vi "Test Load Day.vi"(8 "error in":errorcluster, 10 "Work Folder":path, 11 "Test Data Folder":path) -> (0 "error out":errorcluster, 2 "Report":string, 3 "Passed":bool)   [LabVIEW 2026]
doc: "Tests Load Day.vi on the schema-v2 sample data (Test Data\\Samples, copied into a new case folder and opened with Initialize Stores.vi). The day shown is 2025-10-06, asked for with 17:00 UTC, which holds two sample entries. Checks: two rows and two Day Entries; Row Entry IDs in Start Time order; the ID column of the rows matches Row Entry IDs; project and task names looked up by ID; the Elapsed column (03:45:28 and 00:32:15) and the Description column (the second one empty); Day Entries parallel to the rows.\n\nInputs: Test Data Folder; Work Folder; error in. Outputs: Passed; Report; error out.\n\nGenerated by: Claude"
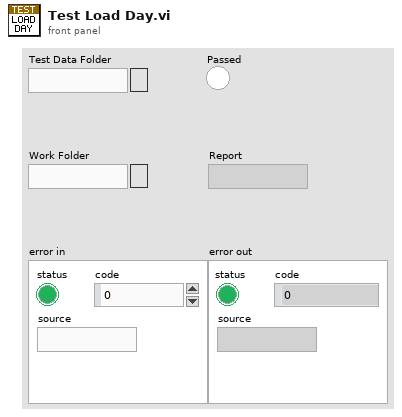
[diagram p1: front panel]
types:
  T1 = typedef "Time Entry List.ctl" = T2[]
  T2 = typedef "Time Entry.ctl" = cluster{"ID":string, "Project ID":string, "Task ID":string, "Start Time":timestamp, "End Time":timestamp, "Description":string}
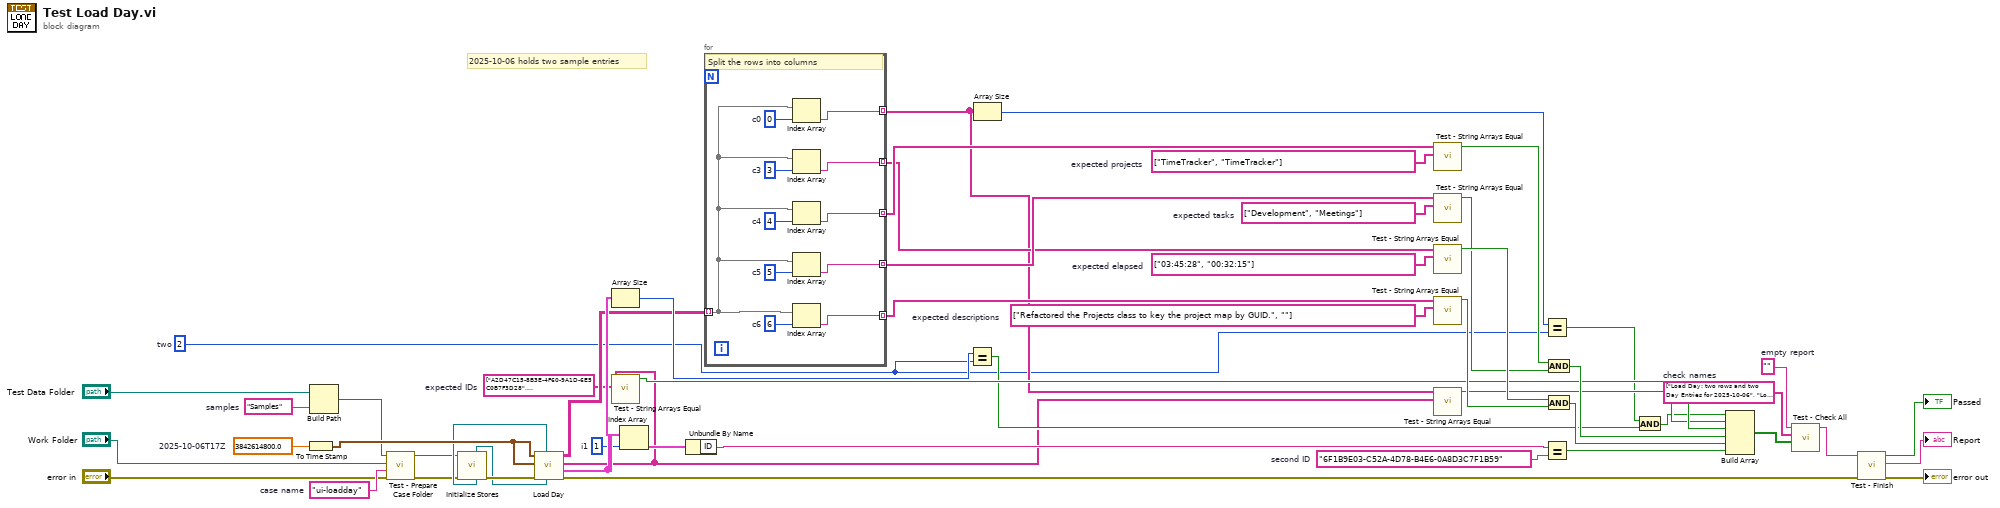
[diagram p0: block diagram]
diagram:
  w19 = string[] ["Load Day: two rows and two Day Entries for 2025-10-06", "Load Day: Row Entry IDs in Start Time order", "Load Day: ID column of the rows matches Row Entry IDs", "Load Day: project and task names looked up by ID", "Load Day: Elapsed and Description columns", "Load Day: Day Entries parallel to the rows"]  # check names
  w18 = string[] ["Refactored the Projects class to key the project map by GUID.", ""]  # expected descriptions
  w17 = string[] ["03:45:28", "00:32:15"]  # expected elapsed
  w16 = string[] ["Development", "Meetings"]  # expected tasks
  w15 = string[] ["TimeTracker", "TimeTracker"]  # expected projects
  w14 = string[] ["A2D47C15-8B3E-4F60-9A1D-6E5C0B7F3D28", "6F1B9E03-C52A-4D78-B4E6-0A8D3C7F1B59"]  # expected IDs
  w13 = "6F1B9E03-C52A-4D78-B4E6-0A8D3C7F1B59"  # second ID
  w12 = 1  # i1
  w11 = 2  # two
  w10 = 3842614800.0  # 2025-10-06T17Z
  w9 = ""  # empty report
  w8 = "ui-loadday"  # case name
  w7 = "Samples"  # samples
  # "2025-10-06 holds two sample entries"
  n1 = To Time Stamp(1:w10) -> (0:w26:timestamp)
  n2 = Build Path(base path="Test Data Folder", name or relative path=w7) -> (appended path=w20:path)
  n3 = call "Test - Prepare Case Folder.vi"("error in (no error)"="error in", "Case Name"=w8, "Work Folder"="Work Folder", "Source Folder"=w20) -> ("error out"=w22:errorcluster, "Case Folder"=w21:path)  [unwired: 6 in]
  n4 = call "Initialize Stores.vi"("error in"=w22, "Data Folder"=w21) -> ("error out"=w25:errorcluster, "Time Entry Store out"=w24:refnum<class "Time Entry Store.lvclass">, "Project Store out"=w23:refnum<class "Project Store.lvclass">)  [unwired: 5 in, 2 out]
  n5 = call "Load Day.vi"("Project Store in"=w23, "Time Entry Store in"=w24, "error in"=w25, "Now"=w26, "Day"=w26) -> ("error out"=w30:errorcluster, "Day Entries"=w29:T1, "Row Entry IDs"=w28:string[], "Rows"=w27:string[][])  [unwired: 1 in, 2 out]
  n6 = Array Size(array=w29) -> (size(s)=w38:i32)
  n7 = call "Test - String Arrays Equal.vi"("Expected"=w14, "Actual"=w28) -> ("Equal?"=w41:bool)  [unwired: 8 in, 1 out]
  n8 = Index Array(array=w29, index=w12) -> (element=w49:T2)
  n9 = Unbundle By Name(w49) -> ("ID"=w50:string)
  n10 = for {
    tunnel: w27 -> [w54] mode=indexing
    tunnel: [w60] -> w31 mode=indexing
    tunnel: [w61] -> w32 mode=indexing
    tunnel: [w62] -> w33 mode=indexing
    tunnel: [w63] -> w34 mode=indexing
    tunnel: [w64] -> w35 mode=indexing
    w59 = 6  # c6
    w58 = 5  # c5
    w57 = 4  # c4
    w56 = 3  # c3
    w55 = 0  # c0
    # "Split the rows into columns"
    n11 = Index Array(array=w54, index=w55) -> (element=w60:string)
    n12 = Index Array(array=w54, index=w56) -> (element=w61:string)
    n13 = Index Array(array=w54, index=w57) -> (element=w62:string)
    n14 = Index Array(array=w54, index=w58) -> (element=w63:string)
    n15 = Index Array(array=w54, index=w59) -> (element=w64:string)
  }
  n16 = Equal?(x=w38, y=w11) -> (x = y?=w39:bool)
  n17 = Array Size(array=w31) -> (size(s)=w36:i32)
  n18 = call "Test - String Arrays Equal.vi"("Expected"=w15, "Actual"=w33) -> ("Equal?"=w43:bool)  [unwired: 8 in, 1 out]
  n19 = call "Test - String Arrays Equal.vi"("Expected"=w16, "Actual"=w34) -> ("Equal?"=w44:bool)  [unwired: 8 in, 1 out]
  n20 = call "Test - String Arrays Equal.vi"("Expected"=w17, "Actual"=w32) -> ("Equal?"=w46:bool)  [unwired: 8 in, 1 out]
  n21 = call "Test - String Arrays Equal.vi"("Expected"=w18, "Actual"=w35) -> ("Equal?"=w47:bool)  [unwired: 8 in, 1 out]
  n22 = call "Test - String Arrays Equal.vi"("Expected"=w28, "Actual"=w31) -> ("Equal?"=w42:bool)  [unwired: 8 in, 1 out]
  n23 = Equal?(x=w36, y=w11) -> (x = y?=w37:bool)
  n24 = Equal?(x=w50, y=w13) -> (x = y?=w51:bool)
  n25 = And(x=w43, y=w44) -> (x .and. y?=w45:bool)
  n26 = And(x=w46, y=w47) -> (x .and. y?=w48:bool)
  n27 = And(x=w37, y=w39) -> (x .and. y?=w40:bool)
  n28 = Build Array(w40, w41, w42, w45, w48, w51) -> (w52:bool[])
  n29 = call "Test - Check All.vi"("Conditions"=w52, "Check Names"=w19, "Report in"=w9) -> ("Report out"=w53:string)  [unwired: 7 in, 1 out]
  n30 = call "Test - Finish.vi"("error in (no error)"=w30, "Report"=w53) -> ("error out"=→"error out":errorcluster, "Report out"=→"Report":string, "Passed"=→"Passed":bool)  [unwired: 7 in]
